vi "Update.vi"(9 "log line":string, 10 "file ref":refnum<file>, 11 "rollover trigger in":refnum<class "RolloverTrigger.Multi.lvclass">) -> (3 "rollover trigger out":refnum<class "RolloverTrigger.Multi.lvclass">)   [LabVIEW 2018, in "GLog.lvlib" / "RolloverTrigger.Multi.lvclass"]
doc: "Updates the internal state of the rollover trigger after the file is written to."
uses:
  RolloverTrigger.Multi.lvclass
  RolloverTrigger.Multi.lvclass/RolloverTrigger.Multi.ctl
  RolloverTrigger/RolloverTrigger.lvclass
panel:
  # "Connector Pane"
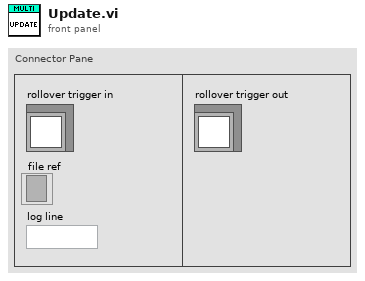
[diagram p1: front panel]
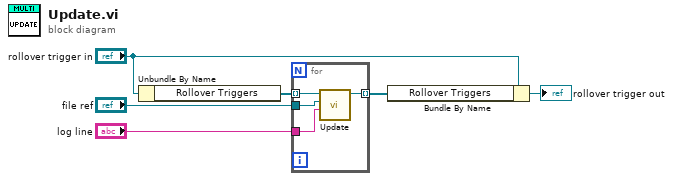
[diagram p0: block diagram]
diagram:
  n1 = Unbundle By Name("rollover trigger in") -> ("Rollover Triggers"=w6:refnum<class "RolloverTrigger.lvclass">[])
  n2 = for {
    tunnel: w6 -> [w10] mode=indexing
    tunnel: [w9] -> w5 mode=indexing
    tunnel: "file ref" -> [w8]
    tunnel: "log line" -> [w7]
    n3 = call-dynamic "Update.vi"("log line"=w7, "file ref"=w8, "rollover trigger in"=w10) -> ("rollover trigger out"=w9:refnum<class "RolloverTrigger.lvclass">)  [unwired: 8 in]
  }
  n4 = Bundle By Name(cluster="rollover trigger in", "Rollover Triggers"=w5) -> (→"rollover trigger out":refnum<class "RolloverTrigger.Multi.lvclass">)
